vi "set Active Window Index.vi"(8 "error in (no error)":errorcluster, 10 "Window":T1, 11 "FSV-40N in":refnum<class "FSV-40N.lvclass">) -> (0 "error out":errorcluster, 3 "FSV-40N out":refnum<class "FSV-40N.lvclass">)   [LabVIEW 2023, in "Spectrum Analyzer.lvlib" / "FSV-40N.lvclass"]
uses:
  FSV-40N.lvclass
  FSV-40N.lvclass/FSV-40N.ctl
  TYPE DEFINITION/TYPE Spectrum Window Select.ctl
  Spectrum Analyzer.lvlib
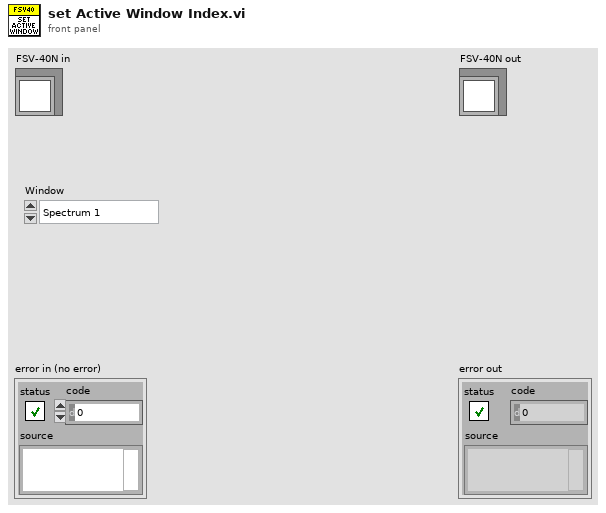
[diagram p1: front panel]
types:
  T1 = typedef "Spectrum Analyzer.lvlib/TYPE Spectrum Window Select.ctl" = enum16{"Spectrum 1", "Spectrum 2", "Spectrum 3", "Spectrum 4"}
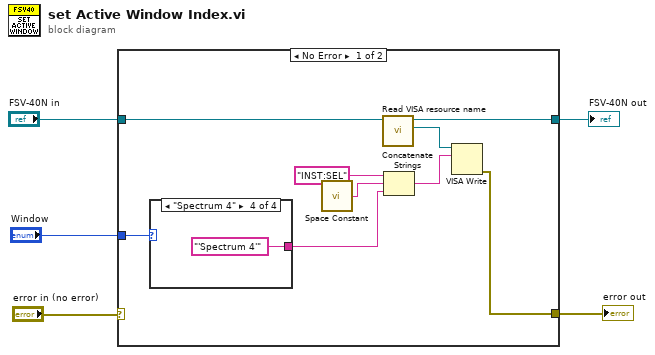
[diagram p0: block diagram]
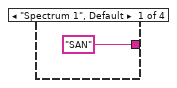
[diagram p2: hidden frame]
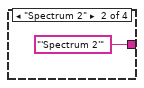
[diagram p3: hidden frame]
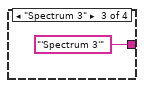
[diagram p4: hidden frame]
diagram:
  n1 = case shown="No Error" "error in (no error)" {
    selector: "error in (no error)" -> [_ w19]
    tunnel: "FSV-40N in" -> [w13 w20]
    tunnel: [w6 w20] -> w4
    tunnel: [w7 w19] -> w2
    tunnel: "Window" -> [w14 _]
    frame No Error {
      n2 = case shown="\"Spectrum 4\"" w14 {
        tunnel: ["SAN" "'Spectrum 2'" "'Spectrum 3'" "'Spectrum 4'"] -> w9
        frame "Spectrum 1", Default {
        }
        frame "Spectrum 2" {
        }
        frame "Spectrum 3" {
        }
        frame "Spectrum 4" {
        }
      }
      n3 = call <vilib>:"Space Constant.vi"() -> ("String"=w10:string)
      n4 = call "Read VISA resource name.vi"("FSV-40N in"=w13) -> ("VISA resource name"=w12:refnum<visa-resource-name>, "FSV-40N out"=w6:refnum<class "FSV-40N.lvclass">)  [unwired: 8 in, 1 out]
      n5 = Concatenate Strings("INST:SEL" ("write buffer"), w10, w9) -> (w8:string)
      n6 = VISA Write(VISA resource name=w12, write buffer=w8) -> (error out=w7:errorcluster)  [unwired: 1 in, 2 out]
    }
    frame Error {
    }
  }
  "error out" <- w2
  "FSV-40N out" <- w4
